vi "Initialize Plot Data.vi"(8 "error in (no error)":errorcluster, 11 "Data Viewer in":refnum<class "Data Viewer.lvclass">) -> (0 "error out":errorcluster, 3 "Data Viewer out":refnum<class "Data Viewer.lvclass">)   [LabVIEW 2020, in "Data Viewer.lvlib" / "Data Viewer.lvclass"]
uses:
  Data Viewer.lvclass
  Data Serie--cluster.ctl
  Plot Property--cluster.ctl
  Data Viewer.lvclass/Data Viewer.ctl
  Data Viewer.lvlib
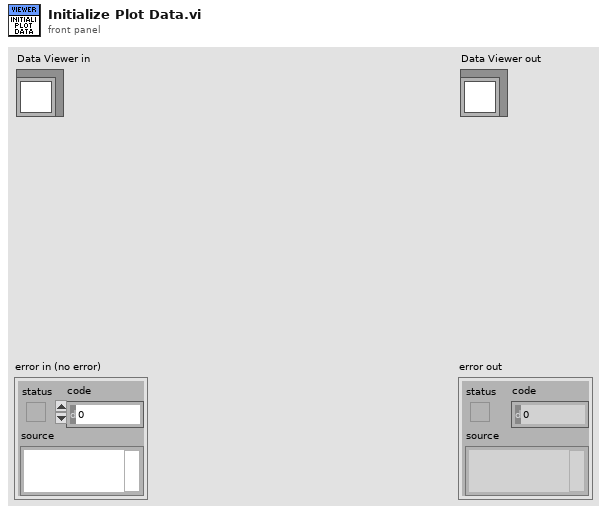
[diagram p1: front panel]
types:
  T1 = typedef "Data Viewer.lvlib/Data Viewer.lvclass/Plot Property--cluster.ctl" = cluster{"Name":string, "Visible":bool, "Color":u32, "Scale Index":i32, "Show Peak Line":bool}
  T2 = typedef "Data Viewer.lvlib/Data Serie--cluster.ctl" = cluster{"Name":string, "Unit":string, "Sample Rate[Hz]":dbl, "Delta t[S]":dbl, "t0":timestamp, "Length":i32, "Time":timestamp[], "Value":dbl[]}
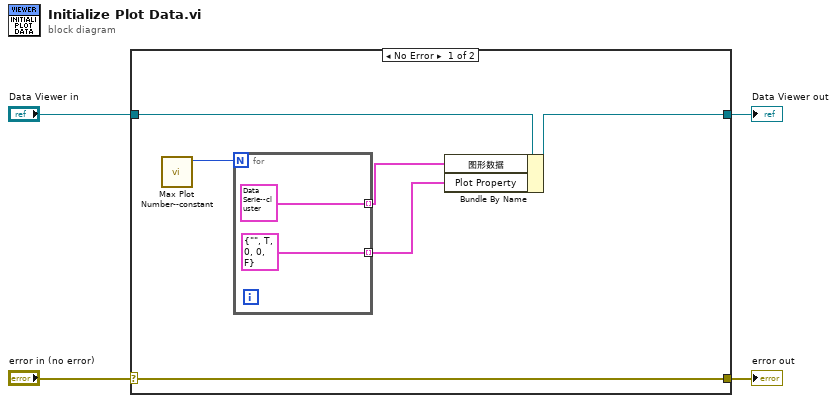
[diagram p0: block diagram]
diagram:
  n1 = case shown="No Error" "error in (no error)" {
    selector: "error in (no error)" -> [w10 w14]
    tunnel: [w10 w14] -> w3
    tunnel: [w6 w13] -> w1
    tunnel: "Data Viewer in" -> [w7 w13]
    frame No Error {
      n2 = call "Max Plot Number--constant.vi"() -> ("Numeric"=w9:i32)  [unwired: 11 in]
      n3 = for {
        N: w9 -> [_]
        tunnel: [T2 {"Name"="", "Unit"="", "Sample Rate[Hz]"=0.0, "Delta t[S]"=0.0, "t0"=timestamp(0 s since 1904-01-01), "Length"=0, "Time"=[], "Value"=[]} ("Data Serie")] -> w8 mode=indexing
        tunnel: [T1 {"Name"="", "Visible"=TRUE, "Color"=0, "Scale Index"=0, "Show Peak Line"=FALSE} ("Plot Property")] -> w5 mode=indexing
      }
      n4 = Bundle By Name(cluster=w7, "图形数据"=w8, "Plot Property"=w5) -> (w6:refnum<class "Data Viewer.lvclass">)
    }
    frame Error {
    }
  }
  "error out" <- w3
  "Data Viewer out" <- w1
